vi "Add-data.vi"(7 "F-UP/T-Down":bool, 10 "Indix":i32=3, 11 "数组":string[][](array[string])=[["1", "3"], ["2", "4"], ["新建表1", ""]]) -> (3 "输出数组":string[][](array[string]))   [LabVIEW 2025]
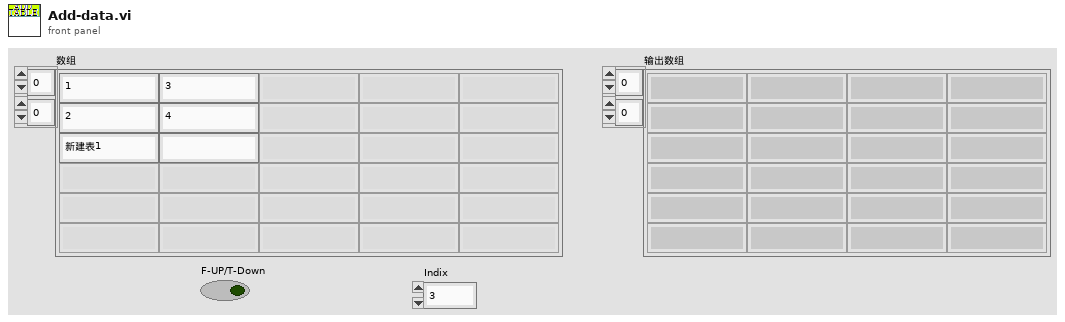
[diagram p1: front panel]
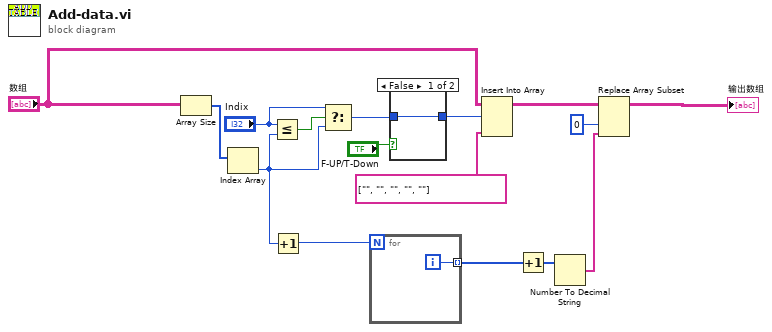
[diagram p0: block diagram]
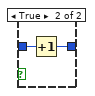
[diagram p2: hidden frame]
diagram:
  n1 = Array Size(array="数组") -> (size(s)=w14:i32[])
  n2 = Index Array(array=w14) -> (element=w8:i32)  [unwired: 1 in]
  n3 = Less Or Equal?(x="Indix", y=w8) -> (x <= y?=w13:bool)
  n4 = Increment(x=w8) -> (x+1=w9:i32)
  n5 = Select(t="Indix", s=w13, f=w8) -> (s? t:f=w3:i32)
  n6 = for {
    N: w9 -> [_]
    tunnel: [w17] -> w7 mode=indexing
    i -> [w17]
  }
  n7 = case shown="False" "F-UP/T-Down" {
    tunnel: w3 -> [w18 w20]
    tunnel: [w18 w19] -> w2
    frame False {
    }
    frame True {
      n8 = Increment(x=w20) -> (x+1=w19:i32)
    }
  }
  n9 = Insert Into Array(array="数组", index (row)=w2, new element=string[] ["", "", "", "", ""]) -> (w11:string[][])  [unwired: 1 in]
  n10 = Increment(x=w7) -> (x+1=w5:i32[])
  n11 = Number To Decimal String(number=w5) -> (decimal integer string=w6:string[])  [unwired: 1 in]
  n12 = Replace Array Subset(array=w11, new element=w6, index (col)=0 ("索引 (行)")) -> (→"输出数组":string[][])  [unwired: 1 in]
